vi "Flatten Waveforms.vi"(8 "error in (no error)":errorcluster, 10 "Waveforms in":waveform(dbl)[](array[waveform])) -> (0 "error out":errorcluster, 1 "flattened data":string, 2 "<JSON> header":string)   [LabVIEW 2019, in "XPUB.lvclass"]
uses:
  XPUB.lvclass
  <vilib>/LabVIEW Open Source Project/Epoch Date & Time/formatter.iso8601/Seconds Units -- enum.ctl
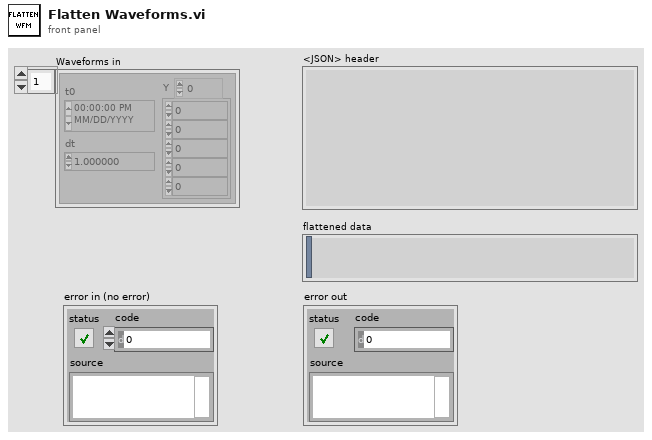
[diagram p1: front panel]
types:
  T1 = typedef "Seconds Units -- enum.ctl" = enum16{"second", "millisecond", "microsecond", "nanosecond"}
  T2 = enum16{"big-endian, network order", "native, host order", "little-endian"}
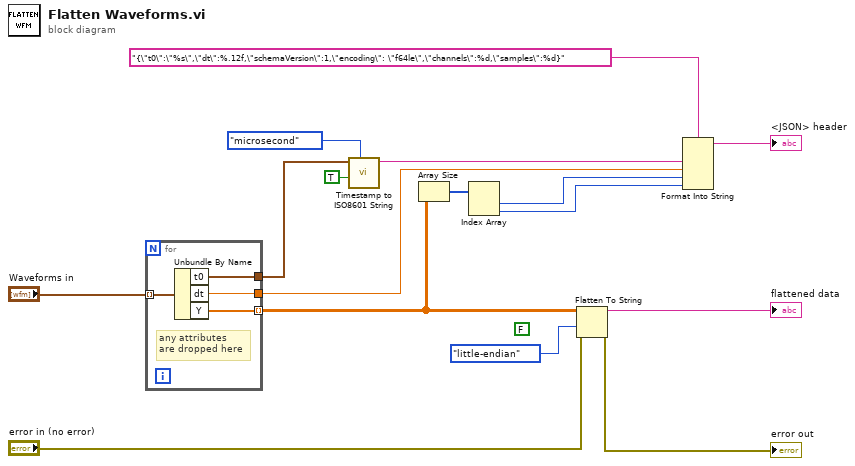
[diagram p0: block diagram]
diagram:
  (unwired) FALSE ("prepend array or string size? (T)")
  n1 = for {
    tunnel: "Waveforms in" -> [w17] mode=indexing
    tunnel: [w20] -> w11 mode=indexing
    tunnel: [w19] -> w14
    tunnel: [w18] -> w3
    # "any attributes\nare dropped here"
    n2 = Unbundle By Name(w17) -> ("t0"=w19:timestamp, "dt"=w18:dbl, "Y"=w20:dbl[])
  }
  n3 = call <vilib>:"Timestamp to ISO8601 String.vi"("Unit (ms)"=Seconds_Units_--_enum."microsecond", "UTC? (F)"=TRUE, "Timestamp (now)"=w14) -> ("ISO8601 String"=w8:string)  [unwired: 8 in]
  n4 = Array Size(array=w11) -> (size(s)=w15:i32[])
  n5 = Index Array(array=w15) -> (element #1=w5:i32, element #2=w4:i32)  [unwired: 2 in]
  n6 = Flatten To String(anything=w11, byte order (0:big-endian, network order)=T2."little-endian", error in (no error)="error in (no error)") -> (data string=→"flattened data":string, error out=→"error out":errorcluster)  [unwired: 1 in, 1 out]
  n7 = Format Into String(format string="{\"t0\":\"%s\",\"dt\":%.12f,\"schemaVersion\":1,\"encoding\": \"f64le\",\"channels\":%d,\"samples\":%d}", w8, w3, w5, w4) -> (resulting string=→"<JSON> header":string)  [unwired: 2 in, 1 out]
